vi "Search and Replace String With Arguments.vi"(8 "error in (no error)":errorcluster, 11 "String":string) -> (0 "error out":errorcluster, 3 "Replaced string":string)   [LabVIEW 2019, in "Error Generation.lvlib"]
doc: "Search in the string-input for <Argument>-strings and replace them with the arguments found in the error cluster.\n\ne.g.\nerror in (no error) has an argument \"delay\" = 1234567\nString = \"The error occured after <daley> seconds\"\n-> Replaced string \"The error occured after 1234567 seconds\"\n- - -\nCopyright (c) 2023, Merecs Engineering GmbH"
uses:
  Error Generation.lvlib
  Is Error Code.vi
  String to Match Pattern Case Insensitive.vi
  <vilib>/Utility/error.llb/Trim Whitespace.vi
panel:
  # "Connector Pane"
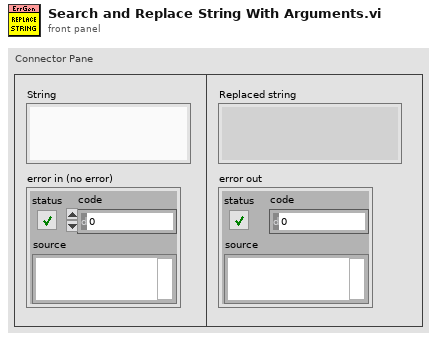
[diagram p1: front panel]
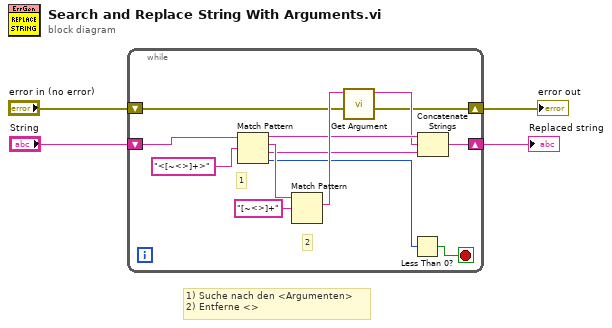
[diagram p0: block diagram]
diagram:
  # "1) Suche nach den <Argumenten>\n2) Entferne <>"
  n1 = while {
    shift-right: [w9] -> w3
    shift-left: "String" -> [w16]
    shift-right: [w5] -> w2
    shift-left: "error in (no error)" -> [w6]
    stop <- w8 stop-if-true
    # "2"
    # "1"
    n2 = Match Pattern(string=w16, regular expression="<[~<>]+>") -> (before substring=w12:string, match substring=w14:string, after substring=w10:string, offset past match=w7:i32)  [unwired: 1 in]
    n3 = Match Pattern(string=w14, regular expression="[~<>]+") -> (match substring=w13:string)  [unwired: 1 in, 3 out]
    n4 = call "Get Argument.vi"("error in (no error)"=w6, "argument"=w13) -> ("error out"=w5:errorcluster, "argument data"=w11:string)  [unwired: 7 in, 1 out]
    n5 = Less Than 0?(x=w7) -> (x < 0?=w8:bool)
    n6 = Concatenate Strings(w12, w11, w10) -> (w9:string)
  }
  "Replaced string" <- w3
  "error out" <- w2
